vi "Process.vi"(8 "error in":errorcluster, 11 "Plugin in":refnum<class "DateTimeChannel.lvclass">) -> (0 "error out":errorcluster, 3 "Plugin out":refnum<class "DateTimeChannel.lvclass">)   [LabVIEW 2023, in "DateTimeChannel.lvlib" / "DateTimeChannel.lvclass"]
uses:
  DateTimeChannel.lvclass
  C:/Program Files/National Instruments/LabVIEW 2023/vi.lib/FlexLogger/SDK/PluginSDK.lvlibp/PEFClasses/SDK/Plugin/Plugin.lvclass
  DateTimeChannel.lvclass/DateTimeChannel.ctl
  <vilib>/FlexLogger/SDK/PluginSDK.lvlibp/PEFClasses/SDK/Plugin/DataHelpers/Write 1D STR (NChan 1 Sample).vi
  <vilib>/FlexLogger/SDK/PluginSDK.lvlibp/PEFClasses/SDK/Plugin/Plugin.lvclass
  C:/Program Files/National Instruments/LabVIEW 2023/vi.lib/FlexLogger/SDK/PluginSDK.lvlibp/PEFClasses/SDK/Processing Element/Processing Element.lvclass
  C:/dev/niflexlogger-plugins/plugins/DateTimeChannel/source/DateTimeChannel/DateTimeChannel.lvclass
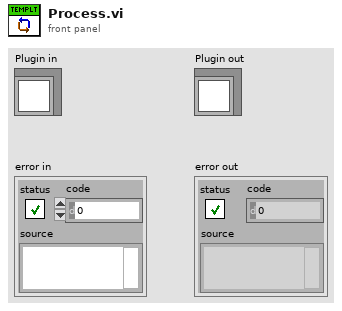
[diagram p1: front panel]
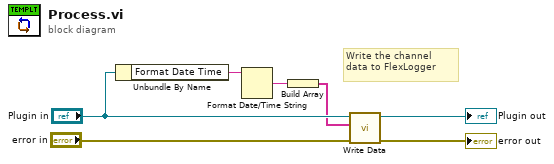
[diagram p0: block diagram]
diagram:
  # "Write the channel data to FlexLogger"
  n1 = Unbundle By Name("Plugin in") -> ("Format Date Time"=w2:string)
  n2 = Format Date/Time String(time format string (%c)=w2) -> (date/time string=w1:string)  [unwired: 2 in]
  n3 = Build Array(w1) -> (w3:string[])
  n4 = call-poly <vilib>:"Write Data.vi"("error in (no error)"="error in", "Data"=w3, "Plugin in"="Plugin in") -> ("error out"=→"error out":errorcluster, "Plugin out"=→"Plugin out":refnum<class "DateTimeChannel.lvclass">)  [unwired: 7 in]
